vi "Get Tree Items.vi"(8 "error in (no error)":errorcluster, 10 "Filter":T1, 11 "Result Model by Reference In":refnum<class "Result Model.lvclass">) -> (0 "error out":errorcluster, 2 "Tree Items":T2(array[cluster]))   [LabVIEW 2020, in "Result Model.lvclass"]
uses:
  Result Model.lvclass
  Tree Item Filter.ctl
  Result Model.lvclass/Result Model.ctl
  Core/Result/Status.ctl
  Core/Result/Result.lvlib
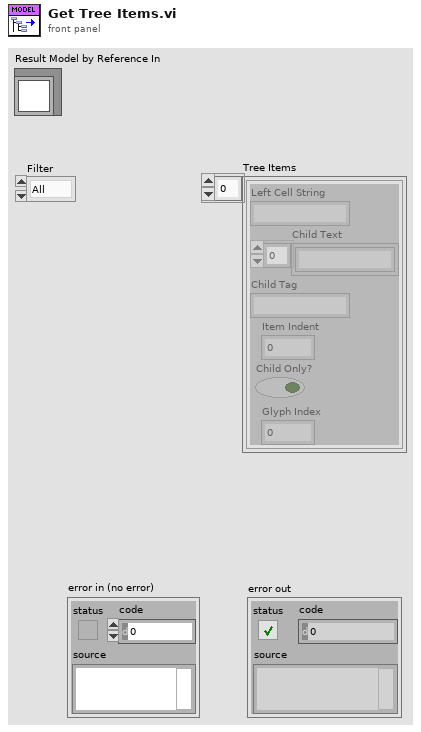
[diagram p1: front panel]
types:
  T1 = typedef "Result Model.lvclass/Tree Item Filter.ctl" = enum16{"All", "Only Fails", "Fails or else Not Executed"}
  T2 = cluster{"Left Cell String":string, "Child Text":string[], "Child Tag":string, "Item Indent":i32, "Child Only?":bool, "Glyph Index":i32}[]
  T3 = typedef "Result.lvlib/Status.ctl" = enum16{"", "Passed", "Failed", "Error", "Skipped", "Setup Error", "Broken", "Teardown Error"}
  T4 = cluster{"Left Cell String":string, "Child Text":string[], "Child Tag":string, "Item Indent":i32, "Child Only?":bool, "Glyph Index":i32}
  T5 = typedef "Result.lvlib/Type.ctl" = enum16{"Test Case", "Test Suite", "Test Run", "Pass", "Fail", "Skip", "Pass if", "Fail if", "Pass if Error", "Fail if Error", "Pass if Equal", "Fail if Equal"}
  T6 = cluster{"Tests":string[], "Run Queue":string[], "Test Statuses":map{string, T3}, "Execution Time":map{string, dbl}, "Assertions":map{string, cluster{"Result Type":T5, "Status":T3, "Description":string, "Data":cluster{"Expected":variant, "Actual":variant, "Delta":variant}}[]}}
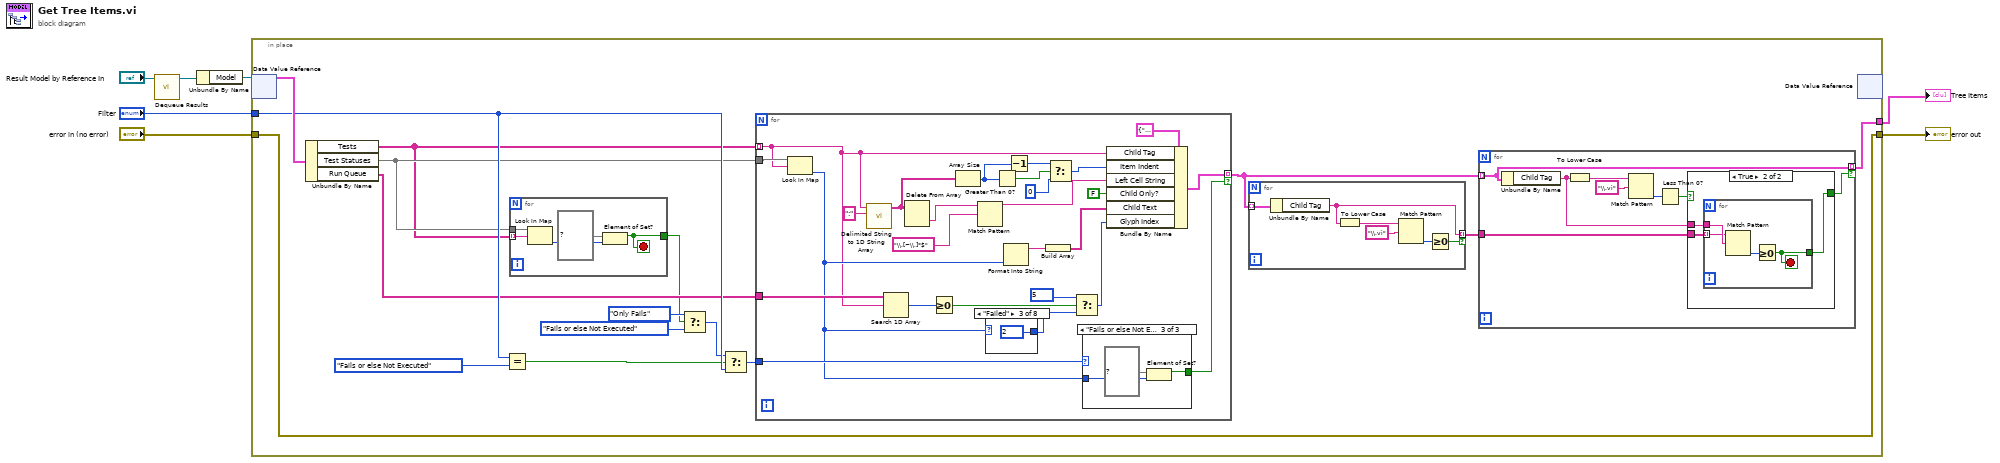
[diagram p0: block diagram]
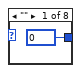
[diagram p2: hidden frame]
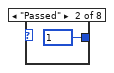
[diagram p3: hidden frame]
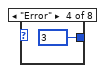
[diagram p4: hidden frame]
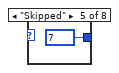
[diagram p5: hidden frame]
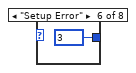
[diagram p6: hidden frame]
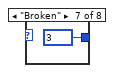
[diagram p7: hidden frame]
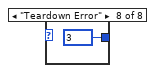
[diagram p8: hidden frame]
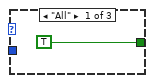
[diagram p9: hidden frame]
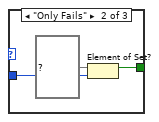
[diagram p10: hidden frame]
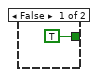
[diagram p11: hidden frame]
diagram:
  n1 = call "Dequeue Results.vi"("Result Model by Reference in"="Result Model by Reference In") -> ("Result Model by Reference out"=w1:refnum<class "Result Model.lvclass">)  [unwired: 10 in]
  n2 = Unbundle By Name(w1) -> ("Model"=w7:refnum<data-value>)
  n3 = in-place {
    in-place-border: "error in (no error)" -> [w23]
    in-place-border: [w23] -> w3
    in-place-border: "Filter" -> [w21]
    in-place-border: [w20] -> w2
    n4 = in-place-dvr #1(w7) -> (w22:T6)  [unwired: 1 out]
    n5 = Unbundle By Name(w22) -> ("Tests"=w18:string[], "Test Statuses"=w19:map{string, T3}, "Run Queue"=w17:string[])
    n6 = Equal?(x=w21, y=Tree_Item_Filter."Fails or else Not Executed") -> (x = y?=w11:bool)
    n7 = for {
      tunnel: [w28] -> w12
      tunnel: w18 -> [w26] mode=indexing
      tunnel: w19 -> [w27]
      stop <- w28 stop-if-true
      n8 = Look In Map(map=w27, key=w26) -> (value=w25:T3)  [unwired: 1 in, 1 out]
      n9 = Element of Set?(10:w25, 11:set{T3} {enum."Failed", enum."Error", enum."Setup Error", enum."Broken", enum."Teardown Error"} ("set out")) -> (3:w28:bool)
    }
    n10 = Select(t=Tree_Item_Filter."Only Fails" ("Filter"), s=w12, f=Tree_Item_Filter."Fails or else Not Executed" ("y")) -> (s? t:f=w15:T1)
    n11 = Select(t=w15, s=w11, f=w21) -> (s? t:f=w9:T1)
    n12 = for {
      tunnel: [w53] -> w8 mode=indexing if=w42
      tunnel: w17 -> [w34]
      tunnel: w9 -> [w43]
      tunnel: w18 -> [w29] mode=indexing
      tunnel: w19 -> [w31]
      n13 = Look In Map(map=w31, key=w29) -> (value=w30:T3)  [unwired: 1 in, 1 out]
      n14 = call <vilib>:"Delimited String to 1D String Array.vi"("delimiter"=":", "delimited string"=w29) -> ("string array"=w49:string[])  [unwired: 9 in]
      n15 = Search 1D Array(1D array=w34, element=w29) -> (index of element=w33:i32)  [unwired: 1 in]
      n16 = Delete From Array(array=w49) -> (deleted portion=w36:string)  [unwired: 2 in, 1 out]
      n17 = Greater Or Equal To 0?(x=w33) -> (x >= 0?=w32:bool)
      n18 = Array Size(array=w49) -> (size(s)=w40:i32)
      n19 = Match Pattern(string=w36, regular expression="\\.[~\\.]*$") -> (before substring=w50:string)  [unwired: 1 in, 3 out]
      n20 = case shown="\"Failed\"" w30 {
        tunnel: [0 ("Listbox Symbol Ring Constant") 1 ("Listbox Symbol Ring Constant") 2 ("Listbox Symbol Ring Constant") 3 ("Listbox Symbol Ring Constant") 7 ("Listbox Symbol Ring Constant") 3 ("Listbox Symbol Ring Constant") 3 ("Listbox Symbol Ring Constant") 3 ("Listbox Symbol Ring Constant")] -> w44
        frame "" {
        }
        frame "Passed" {
        }
        frame "Failed" {
        }
        frame "Error" {
        }
        frame "Skipped" {
        }
        frame "Setup Error" {
        }
        frame "Broken" {
        }
        frame "Teardown Error" {
        }
      }
      n21 = Greater Than 0?(x=w40) -> (x > 0?=w41:bool)
      n22 = Format Into String(w30) -> (resulting string=w48:string)  [unwired: 3 in, 1 out]
      n23 = Decrement(x=w40) -> (x-1=w39:i32)
      n24 = Build Array(w48) -> (w47:string[])
      n25 = Select(t=w39, s=w41, f=0) -> (s? t:f=w38:i32)
      n26 = Select(t=5 ("Listbox Symbol Ring Constant"), s=w32, f=w44) -> (s? t:f=w45:i32)
      n27 = case shown="\"Fails or else Not Executed\"" w43 {
        tunnel: w30 -> [_ w66 w69]
        tunnel: [TRUE w65 w68] -> w42
        frame "All" {
        }
        frame "Only Fails" {
          n28 = Element of Set?(10:w66, 11:set{T3} {enum."Failed", enum."Error", enum."Setup Error", enum."Broken", enum."Teardown Error"} ("set out")) -> (3:w65:bool)
        }
        frame "Fails or else Not Executed" {
          n29 = Element of Set?(10:w69, 11:set{T3} {enum."", enum."Failed", enum."Error", enum."Setup Error", enum."Broken", enum."Teardown Error"} ("set out")) -> (3:w68:bool)
        }
      }
      n30 = Bundle By Name(cluster=T4 {"Left Cell String"="", "Child Text"=[], "Child Tag"="", "Item Indent"=0, "Child Only?"=FALSE, "Glyph Index"=0} ("Item"), "Child Tag"=w29, "Item Indent"=w38, "Left Cell String"=w50, "Child Only?"=FALSE, "Child Text"=w47, "Glyph Index"=w45) -> (w53:T4)
    }
    n31 = for {
      tunnel: w8 -> [w75] mode=indexing
      tunnel: [w70] -> w16 mode=indexing if=w71
      n32 = Unbundle By Name(w75) -> ("Child Tag"=w70:string)
      n33 = To Lower Case(string=w70) -> (all lower case string=w73:string)
      n34 = Match Pattern(string=w73, regular expression="\\.vi") -> (offset past match=w72:i32)  [unwired: 1 in, 3 out]
      n35 = Greater Or Equal To 0?(x=w72) -> (x >= 0?=w71:bool)
    }
    n36 = for {
      tunnel: w8 -> [w83] mode=indexing
      tunnel: [w83] -> w20 mode=indexing if=w76
      tunnel: w16 -> [w77]
      n37 = Unbundle By Name(w83) -> ("Child Tag"=w78:string)
      n38 = To Lower Case(string=w78) -> (all lower case string=w81:string)
      n39 = Match Pattern(string=w81, regular expression="\\.vi") -> (offset past match=w80:i32)  [unwired: 1 in, 3 out]
      n40 = Less Than 0?(x=w80) -> (x < 0?=w79:bool)
      n41 = case shown="True" w79 {
        tunnel: w78 -> [_ w87]
        tunnel: w77 -> [_ w86]
        tunnel: [TRUE w85] -> w76
        frame False {
        }
        frame True {
          n42 = for {
            tunnel: w87 -> [w91]
            tunnel: [w89] -> w85
            tunnel: w86 -> [w88] mode=indexing
            stop <- w89 stop-if-true
            n43 = Match Pattern(string=w88, regular expression=w91) -> (offset past match=w90:i32)  [unwired: 1 in, 3 out]
            n44 = Greater Or Equal To 0?(x=w90) -> (x >= 0?=w89:bool)
          }
        }
      }
    }
    n45 = in-place-dvr #1() -> ()  [unwired: 1 in, 2 out]
  }
  "Tree Items" <- w2
  "error out" <- w3
